vi "Var - Variable Info.vi"(7 "VC Handle":T2=-1, 8 "error in":bool, 11 "name_spec":string) -> (0 "error out":bool, 1 "var type":u32, 2 "alias":string, 3 "var name":string, 4 "has history":bool, 5 "var VC Handle":T2=-1, 6 "err code":T1 items=["No error", "Invalid variable type", "Variable not found", "Variable already exists", "Invalid context handle", "Input error", "Invalid data format", "No history attached", "History already attached", "Invalid history parameters", "Wrong variable name", "Wrong alias name", "Non-unique alias", "Alias not found", "No alias associated", "Alias already associated", "Wrong context name", "Non-unique context name", "Context name not found", "Invalid parameter", "Generic error", "Memory Full", "Unrecognized LV error", "Unknown error code"])   [LabVIEW 2021]
doc: "The VI returns information on a variable. See help for this VI for more information.\n\n<B>VC Handle</B> control has to contain a handle of variable context if <B>name_spec</B> control contains a variable name. In order to get information on a global variable, pass -1 to it. <B>VC Handle</B> is ignored if <B>name_spec</B> refers to a variable by alias.\n\n<B>name_spec</B> control has to contain a name specifier referring to a desired variable. Generic format of a name specifier is\n [name][=alias]\n, where\n 'name' is a variable name.\n 'alias' is an alias associated with a variable; it must follow equal sign (=).\nEither 'name' or '=alias' may be omitted but not both.\n\n::: CalcExpress Toolkit :::\nCopyright (c) 2000-2026 Konstantin Shifershteyn. All rights reserved."
uses:
  cetypes.llb/VarMan Variable Context Handle.ctl
  cetypes.llb/VarMan Error Code.ctl
  cersrc/celveng32.dll
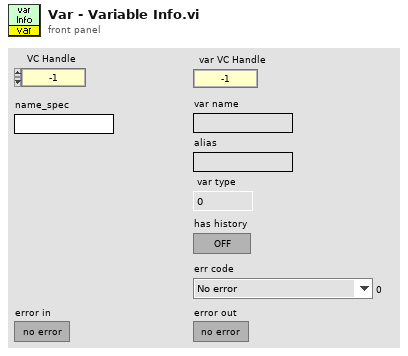
[diagram p1: front panel]
types:
  T1 = typedef "VarMan Error Code.ctl" = u16
  T2 = typedef "VarMan Variable Context Handle.ctl" = i32
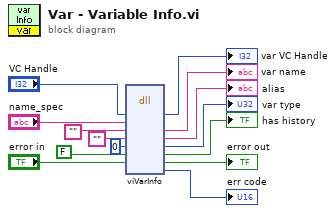
[diagram p0: block diagram]
diagram:
  n1 = dll-call lib="C:/LV Projects/CalcExpress 40 LV2021/vi.lib/addons/CalcExpress/cersrc/celveng*.dll" fn="viVarInfo"("vch"="VC Handle", "nspec"="name_spec", "name"="", "alias"="", "type"=u32 0, "fHist"=FALSE, "errf"="error in") -> ("vch"=→"var VC Handle":T2, "name"=→"var name":string, "alias"=→"alias":string, "type"=→"var type":u32, "fHist"=→"has history":bool, "errf"=→"error out":bool, "err code"=→"err code":T1)  [unwired: 6 in, 2 out]
